vi "Find User in Groups.vi"(4 "error in (no error)":errorcluster, 6 "LoginName":string, 7 "EasyUserManager in":refnum<class "EasyUserManager.lvclass">) -> (0 "error out":errorcluster, 1 "Indexes":i32[](array[numeric]), 2 "Groups":string[](array[string]), 3 "EasyUserManager out":refnum<class "EasyUserManager.lvclass">)   [LabVIEW 2024, in "EasyUserManager.lvclass"]
doc: "Find the user specified by <B>LoginName</B> in all groups. \n\nThis VI returns an array of all group names of which the user is a member and an array of the index of the user in each group."
uses:
  EasyUserManager.lvclass
  EasyUserManager.lvclass/EasyUserManager.ctl
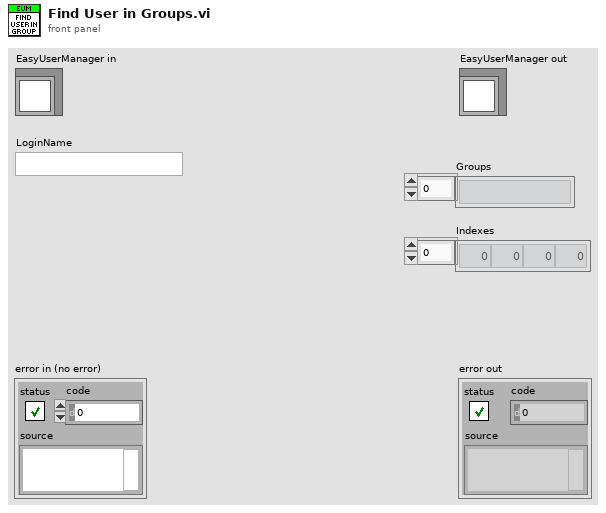
[diagram p1: front panel]
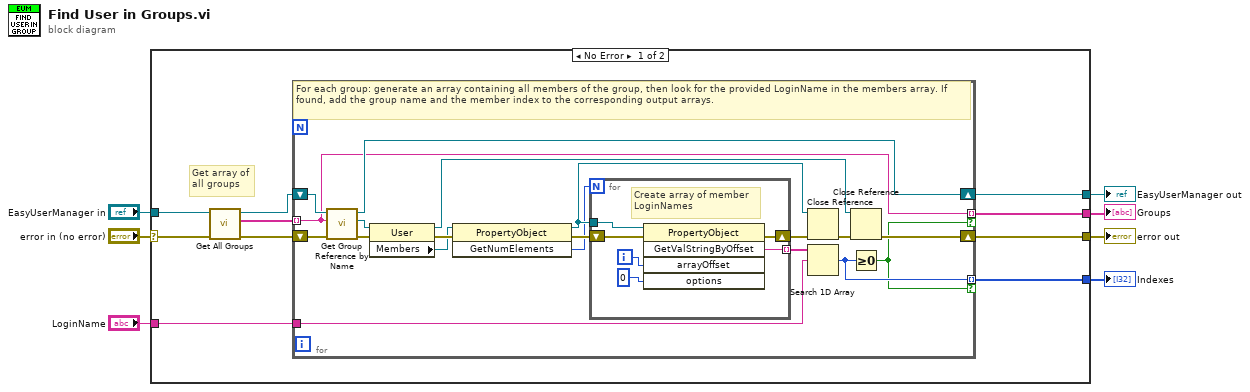
[diagram p0: block diagram]
diagram:
  n1 = case shown="No Error" "error in (no error)" {
    selector: "error in (no error)" -> [w11 w44]
    tunnel: [w13 w44] -> w6
    tunnel: [w14 w43] -> w4
    tunnel: "EasyUserManager in" -> [w17 w43]
    tunnel: "LoginName" -> [w10 _]
    tunnel: [w9 _] -> w2
    tunnel: [w8 _] -> w1
    frame No Error {
      # "Get array of\nall groups"
      n2 = call "Get All Groups.vi"("error in (no error)"=w11, "EasyUserManager in"=w17) -> ("error out"=w15:errorcluster, "Groups"=w12:string[], "EasyUserManager out"=w16:refnum<class "EasyUserManager.lvclass">)  [unwired: 3 in]
      n3 = for {
        shift-right: [w34] -> w14
        shift-left: w16 -> [w36]
        tunnel: w12 -> [w19] mode=indexing
        shift-right: [w23] -> w13
        shift-left: w15 -> [w35]
        tunnel: w10 -> [w22]
        tunnel: [w20] -> w8 mode=indexing if=w18
        tunnel: [w19] -> w9 mode=indexing if=w18
        # "For each group: generate an array containing all members of the group, then look for the provided LoginName in the members array. If found, add the group name and the member index to the corresponding output arrays."
        n4 = call "Get Group Reference by Name.vi"("error in (no error)"=w35, "Group Name"=w19, "EasyUserManager in"=w36) -> ("error out"=w24:errorcluster, "Group Reference"=w21:refnum<k7>, "EasyUserManager out"=w34:refnum<class "EasyUserManager.lvclass">)  [unwired: 2 in]
        n5 = property on="Property Node" class="User"(reference=w21, error in=w24) -> (reference out=w29:refnum<k7>, error out=w27:errorcluster, "Members"=w25:refnum<k7>)
        n6 = invoke on="Invoke Node" class="PropertyObject" method="GetNumElements"(reference=w25, error in=w27) -> (reference out=w33:refnum<k7>, error out=w28:errorcluster, "GetNumElements"=w26:i32)  [unwired: 1 in]
        n7 = for {
          N: w26 -> [_]
          tunnel: w33 -> [w42]
          shift-right: [w38] -> w30
          shift-left: w28 -> [w37]
          tunnel: [w39] -> w32 mode=indexing
          i -> [w40]
          # "Create array of member\nLoginNames"
          n8 = invoke on="Invoke Node" class="PropertyObject" method="GetValStringByOffset"(reference=w42, error in=w37, "arrayOffset"=w40, "options"=0) -> (error out=w38:errorcluster, "GetValStringByOffset"=w39:string)  [unwired: 1 in, 3 out]
        }
        n9 = Close Reference(reference=w33, error in (no error)=w30) -> (error out=w31:errorcluster)
        n10 = Search 1D Array(1D array=w32, element=w22) -> (index of element=w20:i32)  [unwired: 1 in]
        n11 = Close Reference(reference=w29, error in (no error)=w31) -> (error out=w23:errorcluster)
        n12 = Greater Or Equal To 0?(x=w20) -> (x >= 0?=w18:bool)
      }
    }
    frame Error {
      # "Pass error and do nothing."
    }
  }
  "error out" <- w6
  "EasyUserManager out" <- w4
  "Groups" <- w2
  "Indexes" <- w1
